vi "FuncVI-MsgBox2.vi"(5 "InstanceRef":T2, 9 "arg list":T1[](array[typedef]) {"num" format="%.2f"}) -> (0 "error out":bool, 3 "result":T1 {"num" format="%.2f"})   [LabVIEW 2021]
doc: "::: CalcExpress Toolkit :::\nCopyright (c) 2000-2026 Konstantin Shifershteyn. All rights reserved."
uses:
  cetypes.llb/CalcExpress Function Argument Info.ctl
  cetypes.llb/CalcExpress Instance RefNum.ctl
panel:
  in  "max arg num":i32=1000
  in  "min arg num":i32
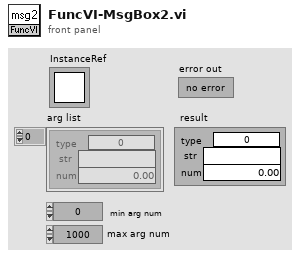
[diagram p1: front panel]
types:
  T1 = typedef "CalcExpress Function Argument Info.ctl" = cluster{"type":u32, "str":string, "num":dbl}
  T2 = typedef "CalcExpress Instance RefNum.ctl" = refnum<k1>
  T3 = enum8{"String", "DBL Number", "identifier", "1D Array of DBL", "2D Array of DBL", "CDB Number", "1D Array of CDB", "2D Array of CDB", "1D Array of String", "2D Array of String", "Unknown data type"}
  T4 = cluster{"type":enum8{"String", "DBL Number", "identifier", "1D Array of DBL", "2D Array of DBL", "CDB Number", "1D Array of CDB", "2D Array of CDB", "1D Array of String", "2D Array of String", "Unknown data type"}, string, dbl}
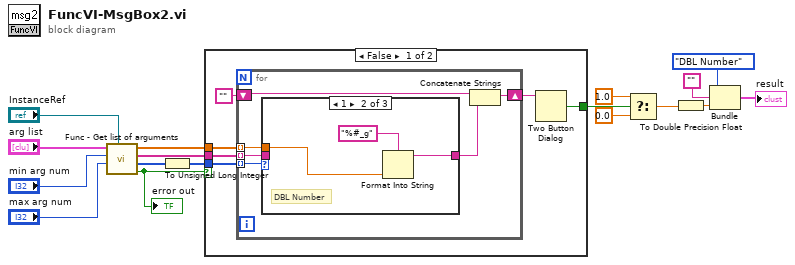
[diagram p0: block diagram]
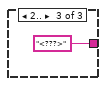
[diagram p3: hidden frame]
diagram:
  n1 = call "Func - Get list of arguments.vi"("InstanceRef"="InstanceRef", "max arg num"="max arg num", "min arg num"="min arg num", "arg list"="arg list") -> ("error out"=w12:bool, "type list"=w15:u32[], "str list"=w16:string[], "num list"=w17:dbl[])  [unwired: 4 in]
  "error out" <- w12
  n2 = To Unsigned Long Integer(number=w15) -> (unsigned 32bit integer=w8:u32[])
  n3 = case shown="False" w12 {
    tunnel: w8 -> [w23 _]
    tunnel: w16 -> [w22 _]
    tunnel: w17 -> [w21 _]
    tunnel: [w18 _] -> w4
    frame False {
      n4 = for {
        tunnel: w21 -> [w27] mode=indexing
        tunnel: w22 -> [w26] mode=indexing
        tunnel: w23 -> [w25] mode=indexing
        shift-right: [w28] -> w19
        shift-left: "" -> [w29]
        n5 = case shown="1" w25 {
          tunnel: [w30 w32 "<???>" ("str")] -> w24
          tunnel: w26 -> [w30 _ _]
          tunnel: w27 -> [_ w31 _]
          frame ..0 {
            # "String"
          }
          frame 1 {
            # "DBL Number"
            n6 = Format Into String(format string="%#_g", w31) -> (resulting string=w32:string)  [unwired: 2 in, 1 out]
          }
          frame 2.. {
          }
        }
        n7 = Concatenate Strings(w29, w24) -> (w28:string)
      }
      n8 = Two Button Dialog(message=w19) -> (T button?=w18:bool)  [unwired: 2 in]
    }
    frame True {
    }
  }
  n9 = Select(t=1.0, s=w4, f=0.0) -> (s? t:f=w3:dbl)
  n10 = To Double Precision Float(number=w3) -> (double precision float=w9:dbl)
  n11 = Bundle("type"=T3."DBL Number", "", w9) -> (→"result":T4)  [unwired: 1 in]
